vi "test add prompt name clash.vi"(8 "error in (no error)":errorcluster, 11 "server id":i32) -> (0 "error out":errorcluster, 3 "body":string)   [LabVIEW 2020, in "MCP Server tests.lvlib"]
doc: "Add Prompt.vi refuses a prompt whose arguments map to the same MCP name. fake prompt name clash.vi has the arguments a b and a_b, which both become a_b: Add Prompt.vi must return error 5010 with a message that names both controls and the MCP name, and must not register the prompt, so prompts/list does not list fake_prompt_name_clash. The 5010 error is cleared after it was checked."
uses:
  MCP Server tests.lvlib
  <vilib>/JDP Science/JSONtext/Next JSON Value.vi
  <vilib>/JDP Science/JSONtext/String Subset.vi
  <vilib>/JDP Science/JSONtext/Parsing/Advance past next JSON Value (inlined COPY).vi
  <vilib>/JDP Science/JSONtext/Parsing/Advance past whitespace.vi
  <vilib>/JDP Science/JSONtext/Parsing/Advance past String.vi
  <vilib>/JDP Science/JSONtext/Parsing/Advance past Number.vi
  <vilib>/JDP Science/JSONtext/Parsing/Advance past Line Ending.vi
  <vilib>/JDP Science/JSONtext/Parsing/Parse Full Path or Item Name.vi
  <vilib>/JDP Science/JSONtext/Parsing/Advance past Array.vi
  <vilib>/JDP Science/JSONtext/Parsing/Advance past Object.vi
  <vilib>/JDP Science/JSONtext/support/Error Cluster From Code.vi
  <vilib>/JDP Science/JSONtext/Offset/Find Item Locations by Path.vi
  <vilib>/addons/_JKI Toolkits/Caraya/classes/Test/Test.lvclass
  src/MCP Server/MCP Server.lvlib
  <vilib>/addons/_JKI Toolkits/Caraya/classes/Assert/Assert.lvclass
  <vilib>/JDP Science/JSONtext/JSONtext.lvlib
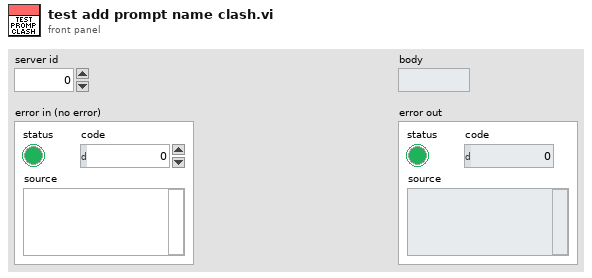
[diagram p1: front panel]
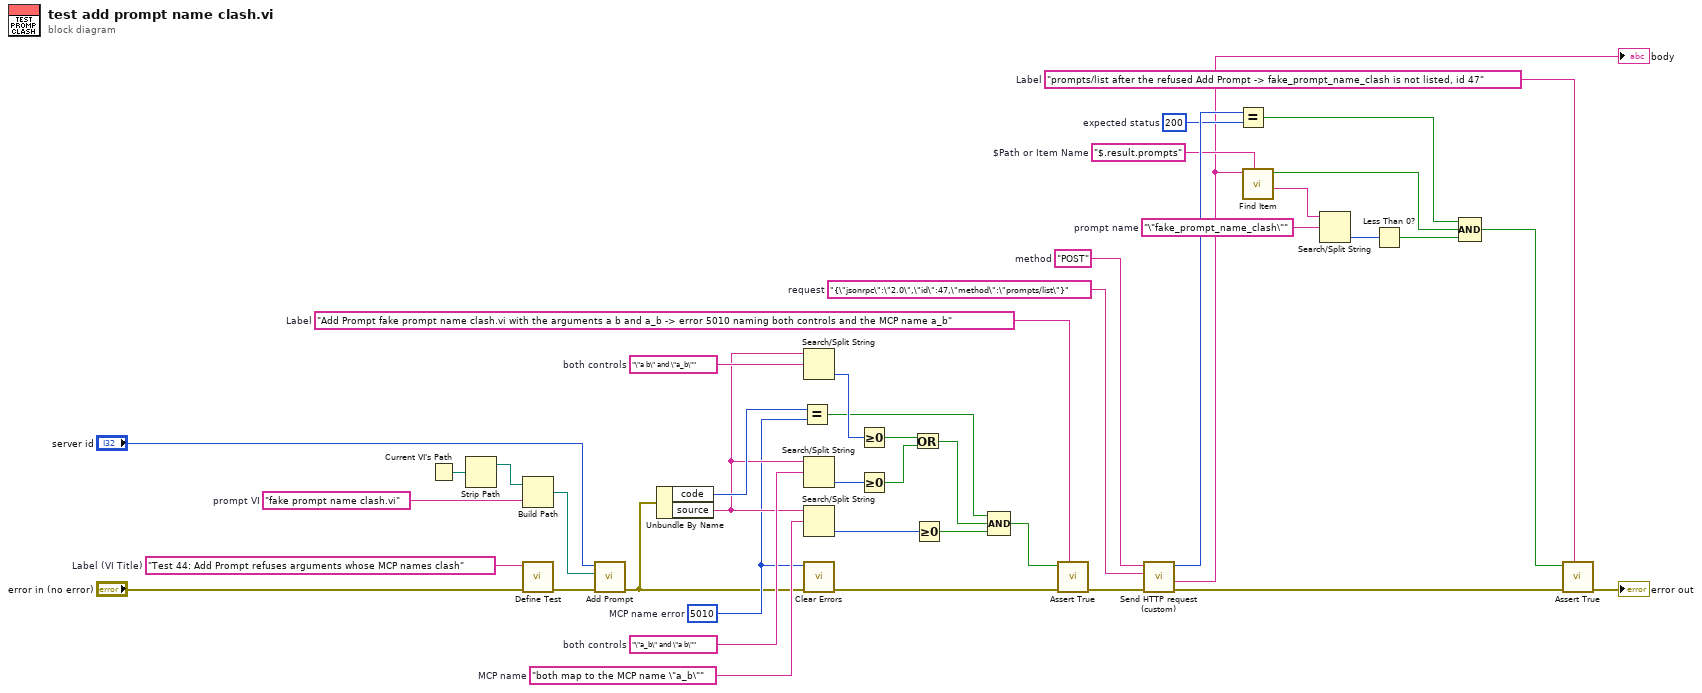
[diagram p0: block diagram]
diagram:
  w3 = "prompts/list after the refused Add Prompt -> fake_prompt_name_clash is not listed, id 47"  # Label
  w10 = "\"fake_prompt_name_clash\""  # prompt name
  w12 = "$.result.prompts"  # $Path or Item Name
  w13 = 200  # expected status
  w16 = "{\"jsonrpc\":\"2.0\",\"id\":47,\"method\":\"prompts/list\"}"  # request
  w17 = "POST"  # method
  w18 = "Add Prompt fake prompt name clash.vi with the arguments a b and a_b -> error 5010 naming both controls and the MCP name a_b"  # Label
  w31 = "both map to the MCP name \"a_b\""  # MCP name
  w33 = "\"a_b\" and \"a b\""  # both controls
  w34 = "\"a b\" and \"a_b\""  # both controls
  w22 = 5010  # MCP name error
  w39 = "fake prompt name clash.vi"  # prompt VI
  w43 = "Test 44: Add Prompt refuses arguments whose MCP names clash"  # Label (VI Title)
  n1 = Current VI's Path() -> (path=w41:path)
  n2 = Strip Path(path=w41) -> (stripped path=w40:path)  [unwired: 1 out]
  n3 = Build Path(base path=w40, name or relative path=w39) -> (appended path=w37:path)
  n4 = call <vilib>:"Define Test.vi"("error in (no error)"="error in (no error)", "Label (VI Title)"=w43) -> ("error out"=w36:errorcluster)  [unwired: 8 in, 1 out]
  n5 = call "Add Prompt.vi"("error in (no error)"=w36, "vi path"=w37, "server id"="server id") -> ("error out"=w21:errorcluster)  [unwired: 7 in, 1 out]
  n6 = Unbundle By Name(w21) -> ("code"=w35:i32, "source"=w32:string)
  n7 = Equal?(x=w35, y=w22) -> (x = y?=w25:bool)
  n8 = Search/Split String(string=w32, search string/char (-)=w34) -> (offset of match=w30:i32)  [unwired: 1 in, 2 out]
  n9 = Search/Split String(string=w32, search string/char (-)=w33) -> (offset of match=w29:i32)  [unwired: 1 in, 2 out]
  n10 = Search/Split String(string=w32, search string/char (-)=w31) -> (offset of match=w28:i32)  [unwired: 1 in, 2 out]
  n11 = call <vilib>:"Clear Errors.vi"("error in (no error)"=w21, "specific error code to clear (0: all)"=w22) -> ("error out"=w19:errorcluster)  [unwired: 4 in, 1 out]
  n12 = Greater Or Equal To 0?(x=w30) -> (x >= 0?=w27:bool)
  n13 = Greater Or Equal To 0?(x=w29) -> (x >= 0?=w26:bool)
  n14 = Or(x=w27, y=w26) -> (x .or. y?=w24:bool)
  n15 = Greater Or Equal To 0?(x=w28) -> (x >= 0?=w23:bool)
  n16 = Compound Arithmetic op=AND(w25, w24, w23) -> (w20:bool)
  n17 = call <vilib>:"Assert True.vi"("Label"=w18, "error in (no error)"=w19, "True?"=w20) -> ("error out"=w15:errorcluster)  [unwired: 7 in, 1 out]
  n18 = call "Send HTTP request (custom).vi"("error in (no error)"=w15, "request"=w16, "method"=w17) -> ("error out"=w4:errorcluster, "response"=w2:string, "status code"=w14:i32)  [unwired: 5 in, 1 out]
  "body" <- w2
  n19 = Equal?(x=w14, y=w13) -> (x = y?=w8:bool)
  n20 = call <vilib>:"Find Item.vi"("$Path or Item Name"=w12, "JSON"=w2) -> ("<JSON>"=w11:string, "Found"=w7:bool)  [unwired: 6 in, 2 out]
  n21 = Search/Split String(string=w11, search string/char (-)=w10) -> (offset of match=w9:i32)  [unwired: 1 in, 2 out]
  n22 = Less Than 0?(x=w9) -> (x < 0?=w6:bool)
  n23 = Compound Arithmetic op=AND(w8, w7, w6) -> (w5:bool)
  n24 = call <vilib>:"Assert True.vi"("Label"=w3, "error in (no error)"=w4, "True?"=w5) -> ("error out"=→"error out":errorcluster)  [unwired: 7 in, 1 out]
